vi "from_string.vi"(8 "error in (no error)":errorcluster, 10 "toml":string, 11 "optional file path (to include in parse error message)":path) -> (0 "error out":errorcluster, 3 "Doc out":refnum<class "Doc.lvclass">)   [LabVIEW 2020, in "toml_edit.lvlib" / "Doc.lvclass"]
uses:
  Doc.lvclass
  Doc.lvclass/Doc.ctl
  dragon_toml_64.dll
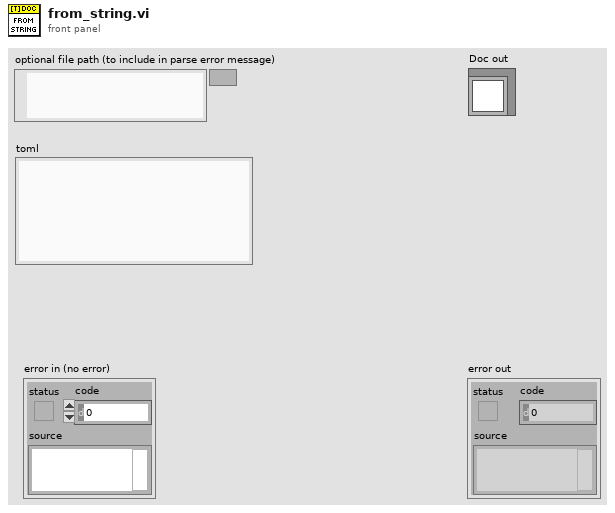
[diagram p1: front panel]
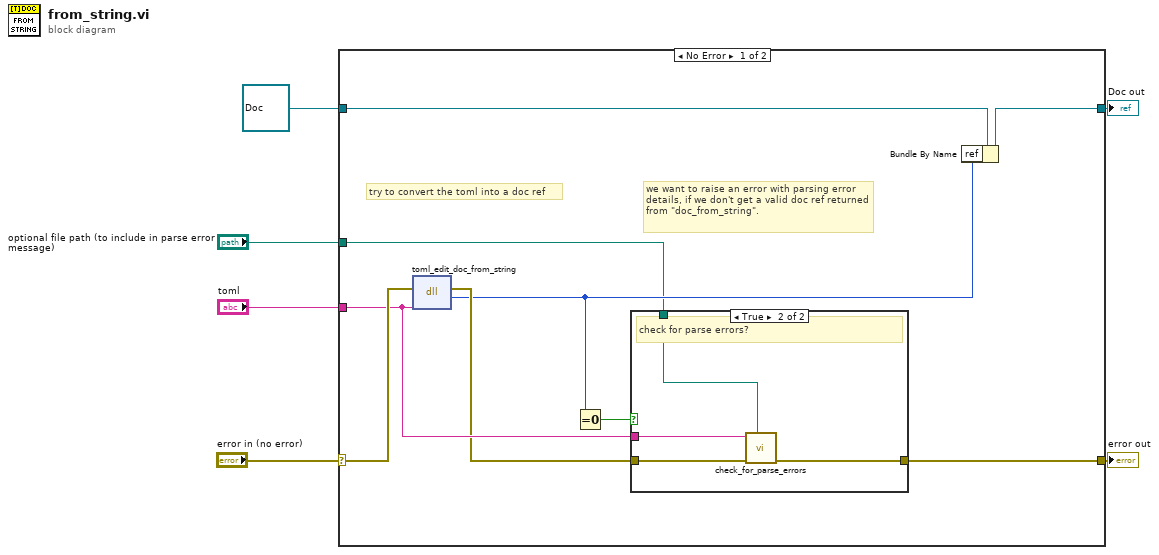
[diagram p0: block diagram]
diagram:
  n1 = case shown="No Error" "error in (no error)" {
    selector: "error in (no error)" -> [w14 w22]
    tunnel: [w10 w22] -> w5
    tunnel: [w13 w21] -> w3
    tunnel: refnum<class "Doc.lvclass"> refnum ("Doc in") -> [w15 w21]
    tunnel: "toml" -> [w12 _]
    tunnel: "optional file path (to include in parse error message)" -> [w7 _]
    frame No Error {
      # "try to convert the toml into a doc ref"
      # "we want to raise an error with parsing error details, if we don't get a valid doc ref returned from \"doc_from_string\"."
      n2 = dll-call lib="C:/projects/dragon-desktop/source/submodules/toml-edit-labview/lv_src/dragon_toml_*.dll" fn="toml_edit_doc_from_string"(error in=w14, "toml_string"=w12) -> (error out=w11:errorcluster, "doc"=w9:u64)  [unwired: 3 in, 1 out]
      n3 = Equal To 0?(x=w9) -> (x = 0?=w8:bool)
      n4 = case shown="True" w8 {
        tunnel: w12 -> [_ w18]
        tunnel: w11 -> [w16 w20]
        tunnel: [w16 w19] -> w10
        tunnel: w7 -> [_ w17]
        frame False {
        }
        frame True {
          # "check for parse errors?"
          n5 = call "check_for_parse_errors.vi"("optional file path (to include in parse error message)"=w17, "error in (no error)"=w20, "toml"=w18) -> ("error out"=w19:errorcluster)  [unwired: 6 in, 2 out]
        }
      }
      n6 = Bundle By Name(cluster=w15, "ref"=w9) -> (w13:refnum<class "Doc.lvclass">)
    }
    frame Error {
    }
  }
  "error out" <- w5
  "Doc out" <- w3
